vi "RemoteVI Drop Closed Clients.vi"(0 "clients":T1(array[cluster])) -> (4 "clients out":T1(array[cluster]))   [LabVIEW 2020, in "RemoteVI.lvlib"]
doc: "Closes the TCP connection of every client marked closed and returns the others, in order. Connections are TCP refnums type-cast to U32."
uses:
  RemoteVI.lvlib
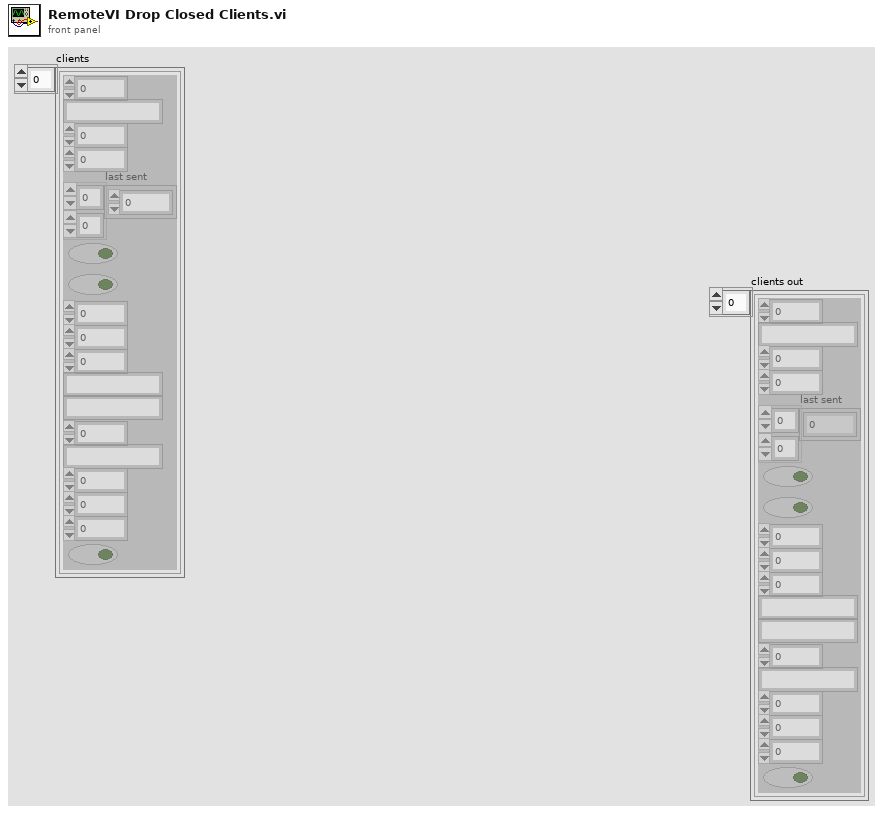
[diagram p1: front panel]
types:
  T1 = cluster{"connection":u32, "rx buffer":string, "seq":u32, "acked":u32, "last sent":u32[][], "tracking":bool, "closed":bool, "mods":u8, "mods set":u8, "popup since":u32, "windows sent":string, "window frames":cluster{"id":u64, "pixels":u32[][]}[], "key window":u64, "address":string, "since":dbl, "last input":dbl, "bytes":dbl, "view only":bool}[]
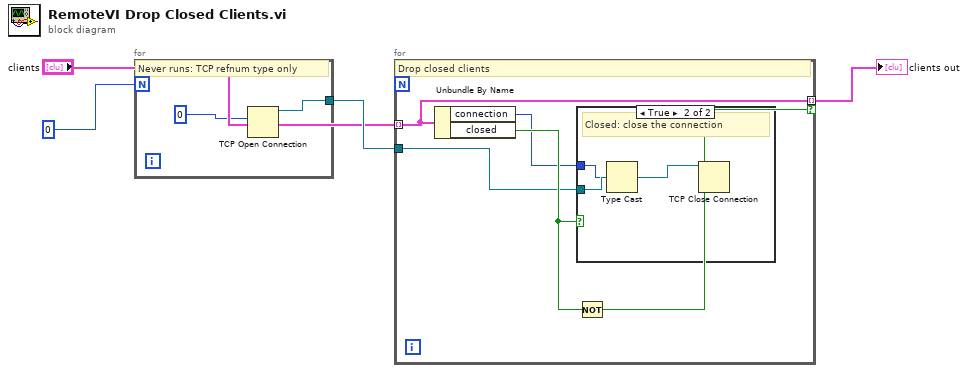
[diagram p0: block diagram]
diagram:
  n1 = for {
    N: 0 -> [_]
    tunnel: [w6] -> w3
    # "Never runs: TCP refnum type only"
    n2 = TCP Open Connection(remote port or service name=u16 0) -> (connection ID=w6:refnum<k5>)  [unwired: 4 in, 1 out]
  }
  n3 = for {
    tunnel: "clients" -> [w7] mode=indexing
    tunnel: [w7] -> w4 mode=indexing if=w11
    tunnel: w3 -> [w8]
    # "Drop closed clients"
    n4 = Unbundle By Name(w7) -> ("connection"=w9:u32, "closed"=w10:bool)
    n5 = case shown="True" w10 {
      tunnel: w9 -> [_ w12]
      tunnel: w8 -> [_ w13]
      frame False {
      }
      frame True {
        # "Closed: close the connection"
        n6 = Type Cast(type=w13, x=w12) -> (*(type *) &x=w14:refnum<k5>)
        n7 = TCP Close Connection(connection ID=w14) -> ()  [unwired: 2 in, 2 out]
      }
    }
    n8 = Not(x=w10) -> (.not. x?=w11:bool)
  }
  "clients out" <- w4
